vi "CIVI Read Frequency Session.vi"(8 "error in":errorcluster, 11 "VISA Session in":refnum<visa-resource-name>="TCPIP0::127.0.0.1::5025::SOCKET") -> (0 "error out":errorcluster, 2 "Frequency (Hz)":i32, 3 "VISA Session out":refnum<visa-resource-name>)   [LabVIEW 2026]
doc: "Queries SENS:FREQ? through an existing VISA session.\nParses the response as an integer frequency in Hz.\nReturns communication and parsing errors.\nDoes not open or close the session."
panel:
  out "Raw Response":string
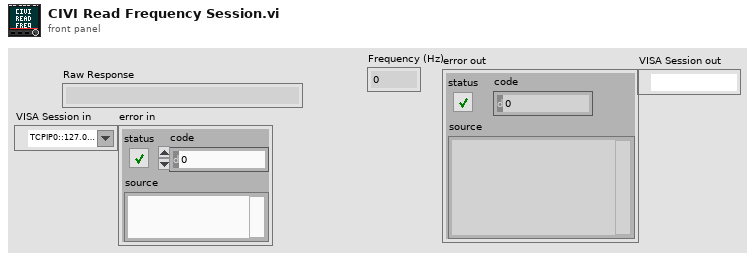
[diagram p1: front panel]
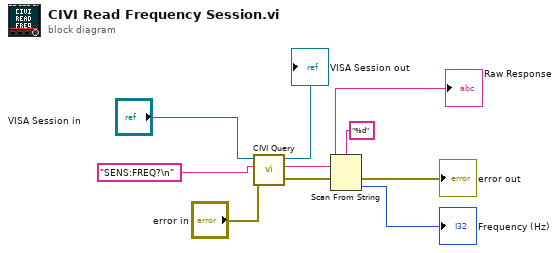
[diagram p0: block diagram]
diagram:
  n1 = call "CIVI Query.vi"("error in"="error in", "write buffer"="SENS:FREQ?\n", "VISA Session in"="VISA Session in") -> ("error out"=w3:errorcluster, "read buffer"=w7:string, "VISA Session out"=→"VISA Session out":refnum<visa-resource-name>)  [unwired: 6 in]
  "Raw Response" <- w7
  n2 = Scan From String(format string="%d", input string=w7, error in=w3) -> (error out=→"error out":errorcluster, output 1=→"Frequency (Hz)":i32)  [unwired: 2 in, 2 out]
